vi "Main.vi"() -> ()   [LabVIEW 2026, in "Application.lvlib"]
doc: "This VI is the main application VI in the DQMH project template. This application VI is implemented as a simple state machine, which communicates with two different DQMH modules.\n_____\nBased on DQMH Dev Tools: Project Template 7.1.2.1547."
uses:
  Application.lvlib
  Application Data--cluster.ctl
  State--enum.ctl
  <vilib>/Utility/error.llb/DialogType.ctl
  <vilib>/Utility/error.llb/Search and Replace Pattern (string).vi
  My Cloneable Module/My Cloneable Module.lvlib
  testCoordinator/testCoordinator.lvlib
panel:
  in  "Start Test Procedure":bool
  out "element":string
  in  "Multicolumn Listbox":i32(listbox)
  in  "About DQMH":bool
  out "version":string
  in  "Hide My Singleton Module":bool
  in  "Show My Singleton Module":bool
  in  "Hide My Cloneable Module":bool
  in  "Show My Cloneable Module":bool
  in  "Stop My Cloneable Module":bool
  in  "Stop My Singleton Module":bool
  in  "Start My Singleton Module":bool
  out "Active Cloneable Modules":string[](array[string])
  in  "Start New Instance My Cloneable Module":bool
  in  "Select Cloneable Module Instance":i32(ring)=-1 items=["All"=-1]
  in  "My Singleton Module: Do Something Else":dbl caption="Do Something Else"
  in  "My Singleton Module: Do Something":bool
  out "My Singleton Running?":bool
  out "Status":string
  in  "My Cloneable Module: Do Something Else":dbl caption="Do Something Else to Selected Module"
  in  "My Cloneable Module: Do Something":bool caption="Do Something to Selected Module"
  # "This top-level application allows you to launch and control a singleton module, and multiple instances of a cloneable module."
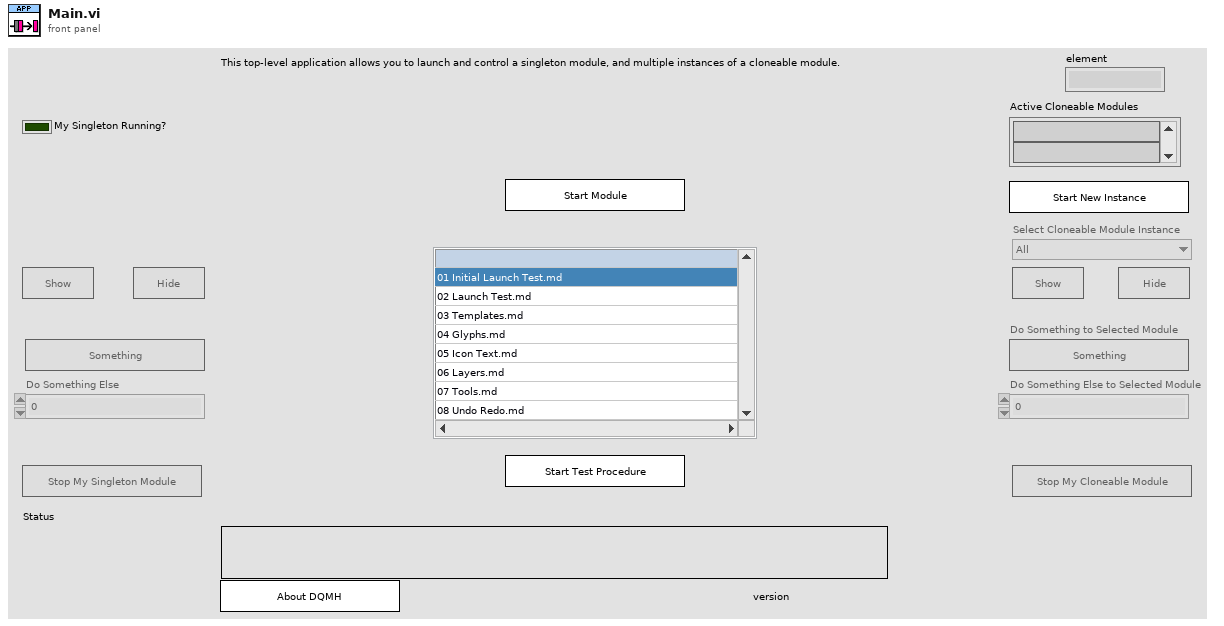
[diagram p1: front panel]
types:
  T1 = typedef "Application.lvlib/State--enum.ctl" = enum16{"Initialize", "Initialize Panel", "UI Interlocks", "Update Status", "Wait for Event", "Exit"}
  T2 = typedef "Application.lvlib/Application Data--cluster.ctl" = cluster{"Status":string, "Singleton Controls":refnum<vi>[], "Cloneable Controls":refnum<vi>[], "Module Ring Value":i32}
  T3 = typedef "My Cloneable Module.lvlib/Broadcast Events--cluster.ctl" = cluster{"Module Did Init":refnum<user-event>, "Status Updated":refnum<user-event>, "Error Reported":refnum<user-event>, "Did Something":refnum<user-event>, "Module Did Stop":refnum<user-event>, "Update Module Execution Status":refnum<user-event>}
  T4 = typedef "testCoordinator.lvlib/Broadcast Events--cluster.ctl" = cluster{"Module Did Init":refnum<user-event>, "Status Updated":refnum<user-event>, "Error Reported":refnum<user-event>, "Did Something":refnum<user-event>, "Module Did Stop":refnum<user-event>, "Update Module Execution Status":refnum<user-event>, "Broadcast Available Tests":refnum<user-event>, "Refresh Test Procedure Indicator":refnum<user-event>, "Refresh Section Indicator":refnum<user-event>, "Refresh Instruction Indicator":refnum<user-event>, "Broadcast Test Scope":refnum<user-event>, "Broadcast Actual Test Procedure Section":refnum<user-event>}
  T5 = enum8{"Enabled", "Disabled", "Disabled and Grayed Out"}
  T6 = typedef "DialogType.ctl" = u16
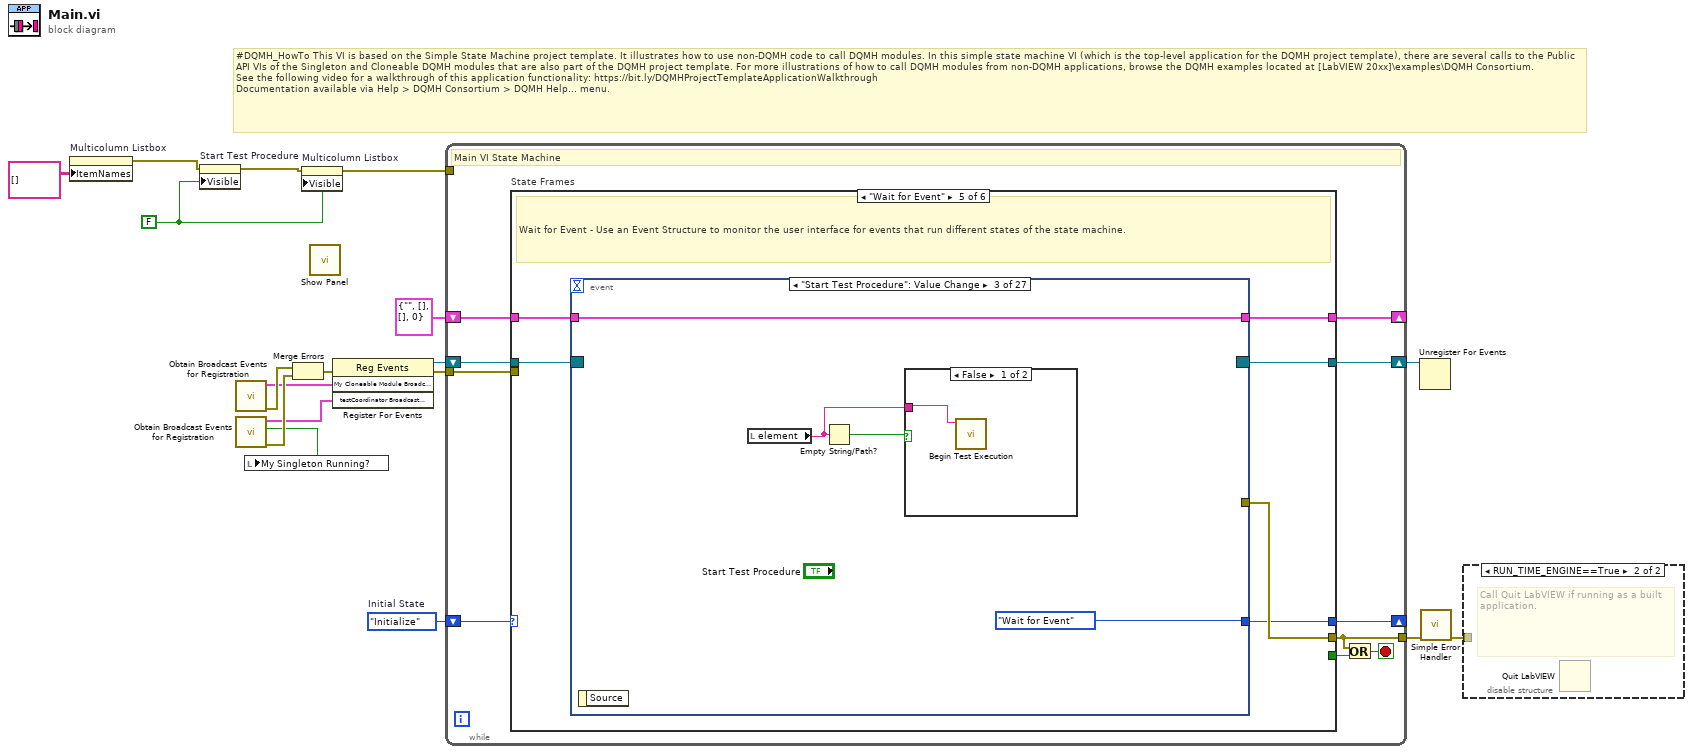
[diagram p0: block diagram]
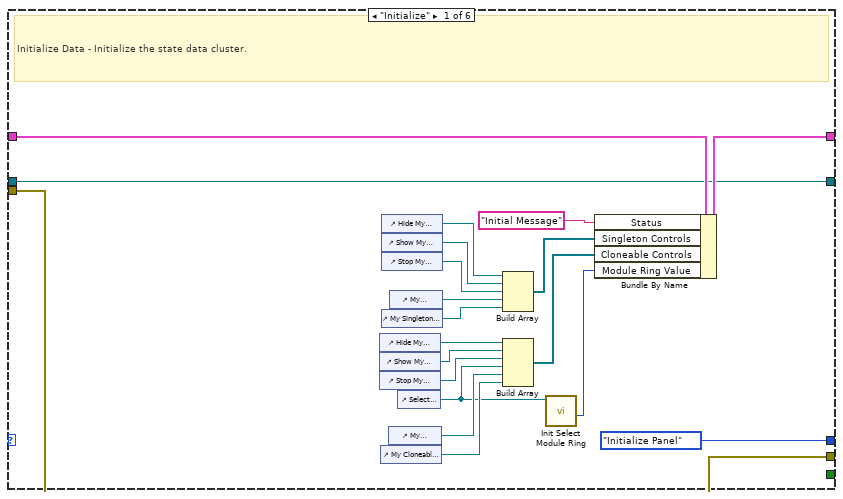
[diagram p2: hidden frame]
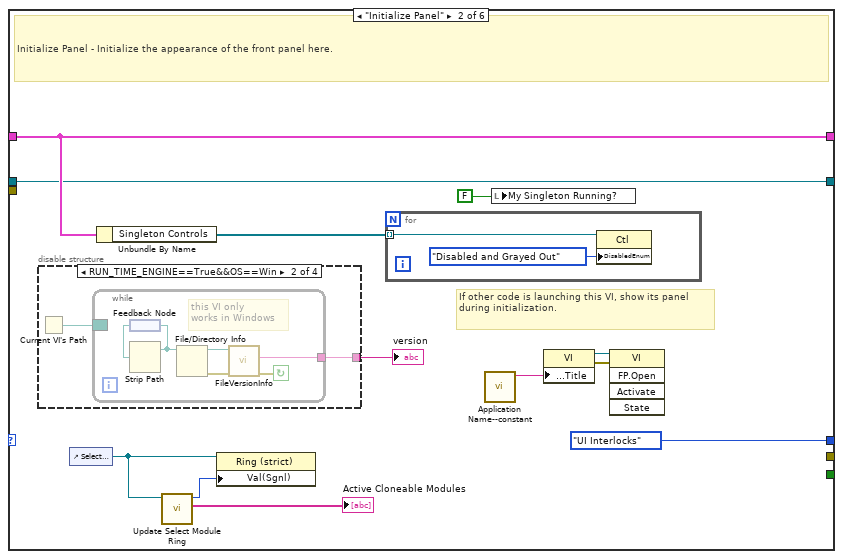
[diagram p3: hidden frame]
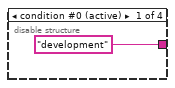
[diagram p4: hidden frame]
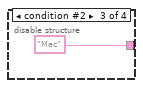
[diagram p5: hidden frame]
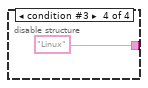
[diagram p6: hidden frame]
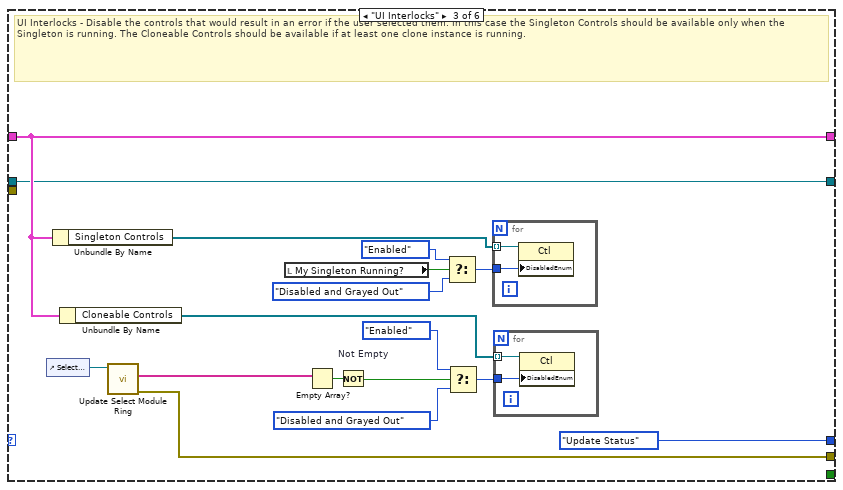
[diagram p7: hidden frame]
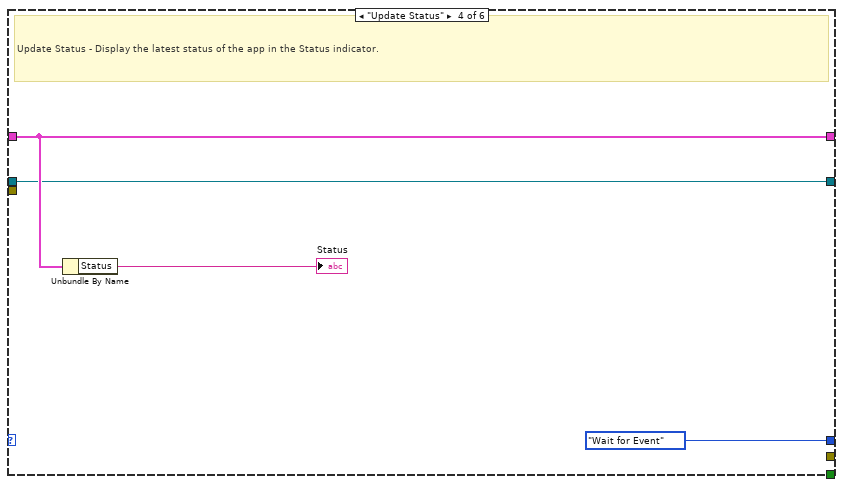
[diagram p8: hidden frame]
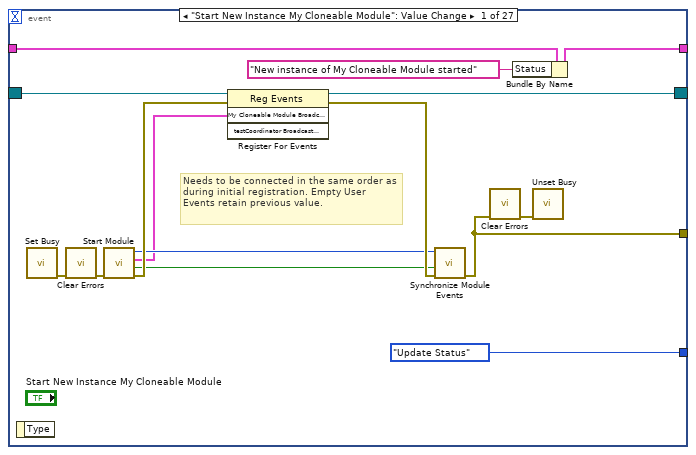
[diagram p9: hidden frame]
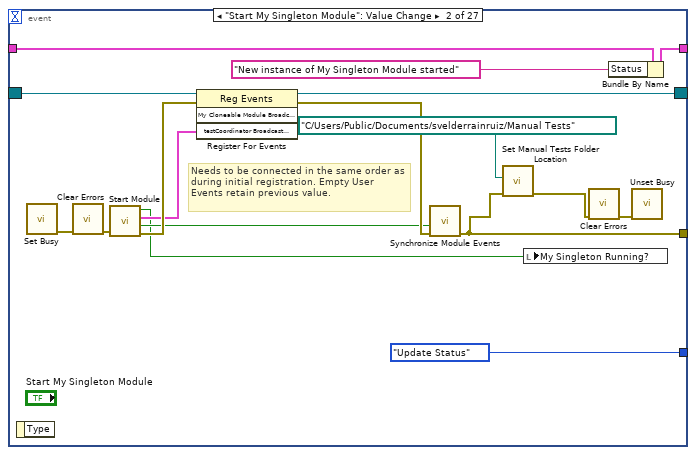
[diagram p10: hidden frame]
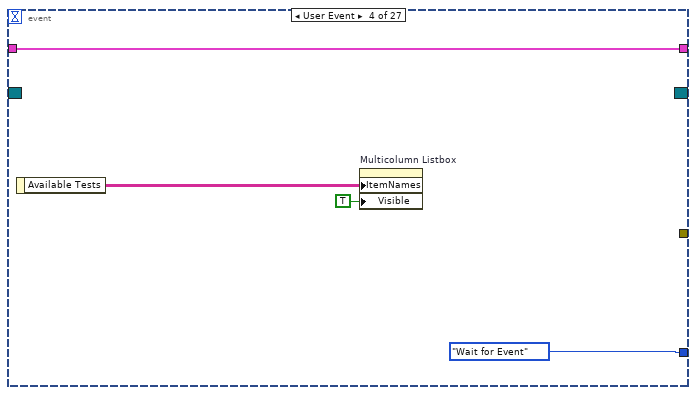
[diagram p12: hidden frame]
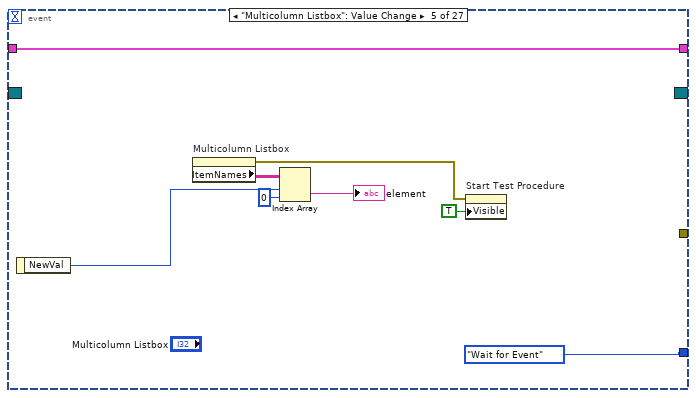
[diagram p13: hidden frame]
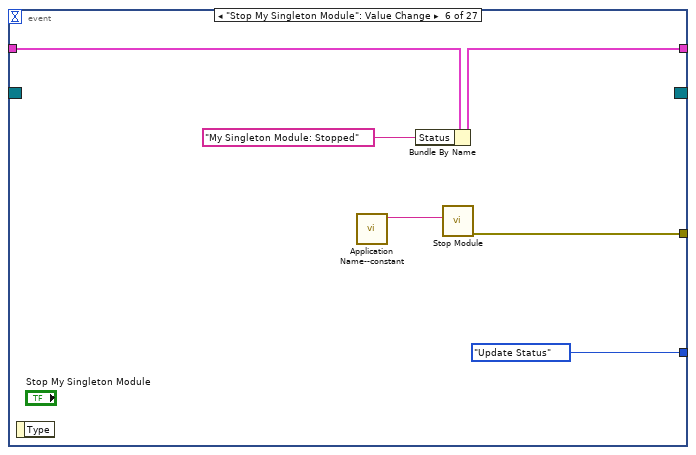
[diagram p14: hidden frame]
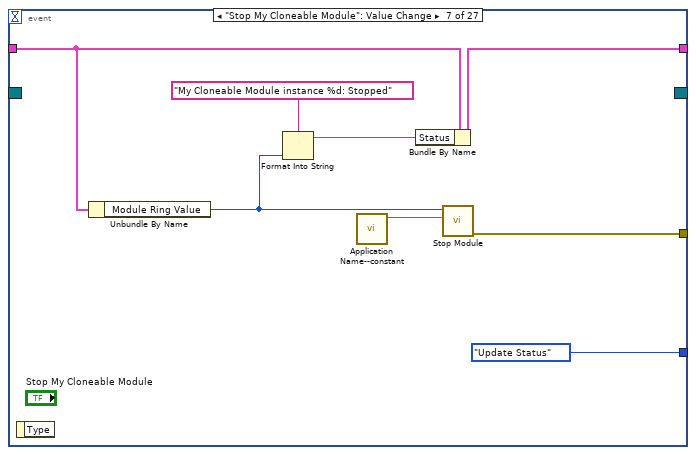
[diagram p15: hidden frame]
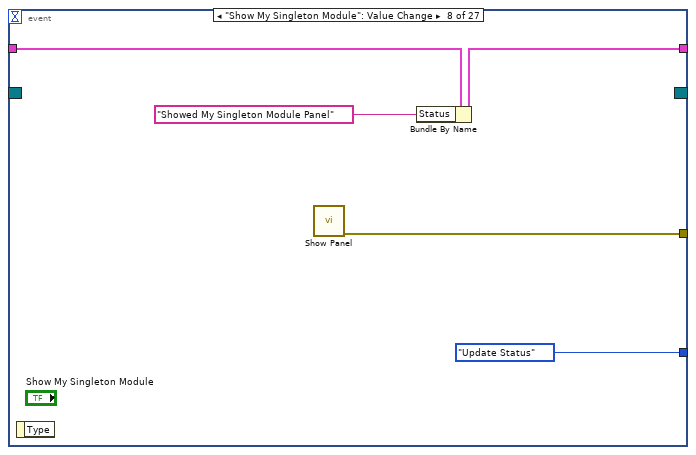
[diagram p16: hidden frame]
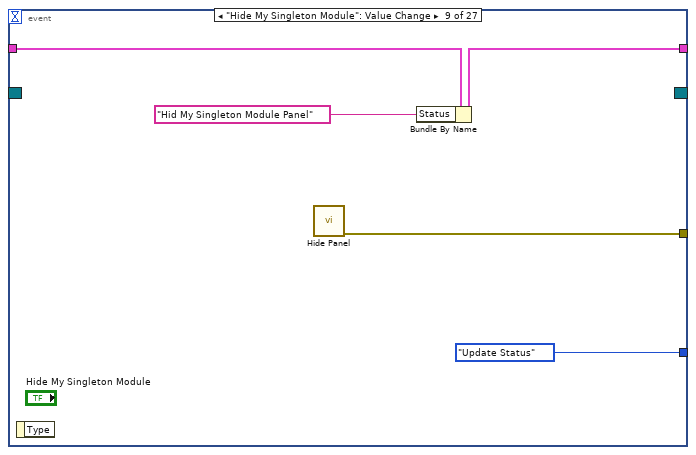
[diagram p17: hidden frame]
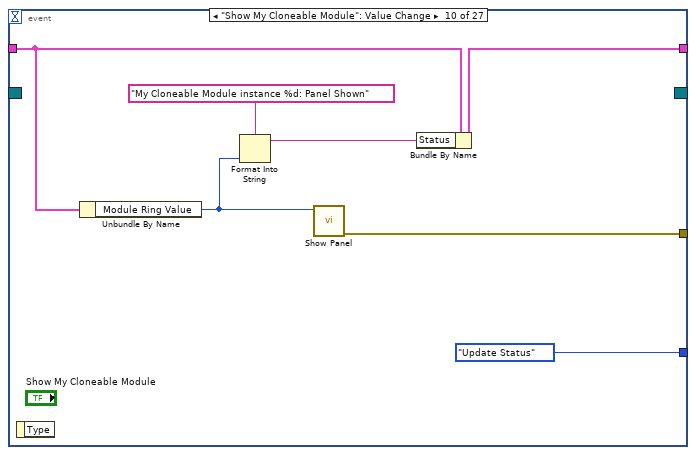
[diagram p18: hidden frame]
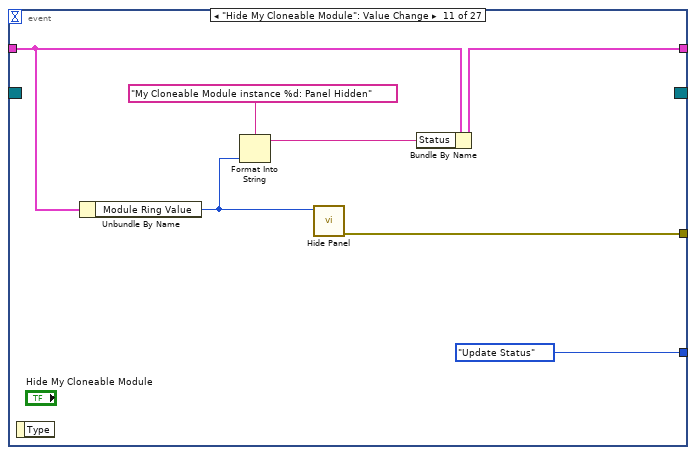
[diagram p19: hidden frame]
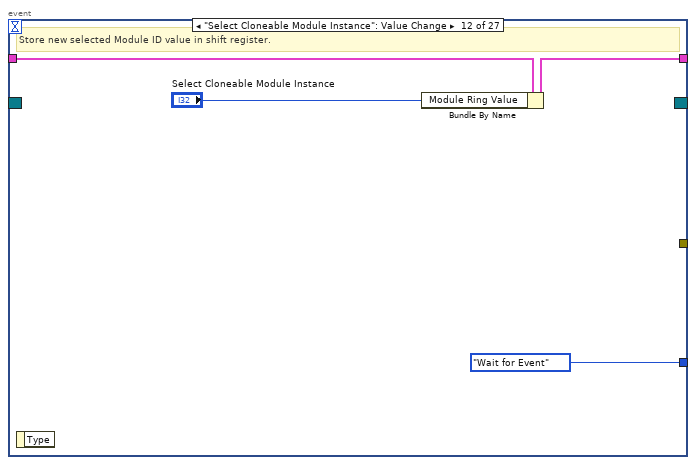
[diagram p20: hidden frame]
diagram:
  w3 = FALSE ("Visible")
  w9 = State--enum."Initialize"  # Initial State
  # "#DQMH_HowTo This VI is based on the Simple State Machine project template. It illustrates how to use non-DQMH code to call DQMH modules. In this simple state machine VI (which is the top-level application for the DQMH project template), there are several calls to the Public API VIs of the Singleton and Cloneable DQMH modules that are also part of the DQMH project template. For more illustrations of how to call DQMH modules from non-DQMH applications, browse the DQMH examples located at [LabVIEW 20xx]\\examples\\DQMH Consortium.\nSee the following video for a walkthrough of this application functionality: https://bit.ly/DQMHProjectTemplateApplicationWalkthrough\nDocumentation available via Help > DQMH Consortium > DQMH Help... menu."
  n1 = property on="Multicolumn Listbox" class="MCListbox (strict)"("ItemNames"=string[][] [] ("Item Names")) -> (error out=w2:errorcluster)  [unwired: 2 in, 1 out]
  n2 = property on="Start Test Procedure" class="Bool"(error in=w2, "Visible"=w3) -> (error out=w4:errorcluster)  [unwired: 1 in, 1 out]
  n3 = call "Obtain Broadcast Events for Registration.vi"() -> ("error out"=w14:errorcluster, "My Cloneable Module Broadcast Events"=w11:T3)  [unwired: 9 in, 1 out]
  n4 = call "Obtain Broadcast Events for Registration.vi"() -> ("error out"=w13:errorcluster, "Already running?"=w6:bool, "testCoordinator Broadcast Events"=w10:T4)  [unwired: 9 in]
  n5 = local write "My Singleton Running?"(w6) -> ()
  n6 = Merge Errors(w14, w13) -> (w15:errorcluster)
  n7 = property on="Multicolumn Listbox" class="MCListbox (strict)"(error in=w4, "Visible"=w3) -> (error out=w5:errorcluster)  [unwired: 1 in, 1 out]
  n8 = call "Show Panel.vi"() -> ()  [unwired: 11 in, 1 out]
  n9 = register-events(error in=w15, w11, w10) -> (reference out=w8:refnum<event-registration>, error out=w16:errorcluster)  [unwired: 1 in]
  n10 = while {
    shift-right: [w25] -> _
    shift-left: T2 {"Status"="", "Singleton Controls"=[], "Cloneable Controls"=[], "Module Ring Value"=0} ("Data Cluster") -> [w26]
    tunnel: [w28] -> w18
    shift-right: [w21] -> _
    shift-left: w9 -> [w23]
    shift-right: [w19] -> w7
    shift-left: w8 -> [w20]
    tunnel: w16 -> [w27]
    tunnel: w5 -> [_]
    stop <- w22 stop-if-true
    # "Main VI State Machine"
    n11 = case "State Frames" shown="\"Wait for Event\"" w23 {
      tunnel: [w48 _ w90 _ w104 w301] -> w28
      tunnel: w26 -> [w47 w57 w78 w98 w101 w298]
      tunnel: [w46 w57 w78 w98 w100 w298] -> w25
      tunnel: [_ _ _ _ _ w297] -> w24
      tunnel: [State--enum."Initialize Panel" ("State") State--enum."UI Interlocks" ("State") State--enum."Update Status" ("State") State--enum."Wait for Event" ("State") w99 State--enum."Exit" ("State")] -> w21
      tunnel: w20 -> [w29 w54 w74 w95 w103 w295]
      tunnel: [w29 w54 w74 w95 w102 w295] -> w19
      tunnel: w27 -> [w48 _ _ _ _ _]
      frame "Initialize" {
        # "Initialize Data - Initialize the state data cluster."
        n12 = control-ref of="Hide My Cloneable Module"() -> (w38:refnum<vi>)
        n13 = control-ref of="Show My Cloneable Module"() -> (w37:refnum<vi>)
        n14 = control-ref of="Stop My Cloneable Module"() -> (w36:refnum<vi>)
        n15 = control-ref of="My Cloneable Module: Do Something"() -> (w33:refnum<vi>)
        n16 = control-ref of="Hide My Singleton Module"() -> (w44:refnum<vi>)
        n17 = control-ref of="Show My Singleton Module"() -> (w43:refnum<vi>)
        n18 = control-ref of="Stop My Singleton Module"() -> (w42:refnum<vi>)
        n19 = control-ref of="My Singleton Module: Do Something"() -> (w40:refnum<vi>)
        n20 = control-ref of="My Cloneable Module: Do Something Else"() -> (w34:refnum<vi>)
        n21 = control-ref of="My Singleton Module: Do Something Else"() -> (w41:refnum<vi>)
        n22 = control-ref of="Select Cloneable Module Instance"() -> (w31:refnum<vi>)
        n23 = Build Array(w44, w43, w42, w41, w40) -> (w39:refnum<vi>[])
        n24 = Build Array(w38, w37, w36, w31, w34, w33) -> (w35:refnum<vi>[])
        n25 = call "Init Select Module Ring.vi"("Select Module Ring Ref"=w31) -> ("Module Ring Value"=w30:i32)  [unwired: 8 in, 2 out]
        n26 = Bundle By Name(cluster=w47, "Status"="Initial Message" ("Initial Message"), "Singleton Controls"=w39, "Cloneable Controls"=w35, "Module Ring Value"=w30) -> (w46:T2)
      }
      frame "Initialize Panel" {
        # "If other code is launching this VI, show its panel during initialization."
        # "Initialize Panel - Initialize the appearance of the front panel here."
        n27 = disable-structure "Conditional Disable Structure" shown="RUN_TIME_ENGINE==True&&OS==Win" {
          disable-tunnel: ["development" w62 "Mac" "Linux"] -> w51
          frame condition #0 (active) {
          }
          frame condition #1 {
            n28 = Current VI's Path() -> (path=w63:path)
            n29 = while {
              border: w63 -> [_]
              tunnel: [w64] -> w62
              stop <- w68 continue-if-true
              # "this VI only \nworks in Windows"
              n30 = feedback #1() -> (w67:path)
              n31 = Strip Path(path=w67) -> (stripped path=w66:path)  [unwired: 1 out]
              n32 = feedback-in #1(w66) -> ()
              n33 = File/Directory Info(path=w66) -> (path out=w65:path, error out=w69:errorcluster)  [unwired: 1 in, 5 out]
              n34 = call <vilib>:"FileVersionInfo.vi"("error in (no error)"=w69, "Application Path in"=w65) -> ("error out"=w68:errorcluster, "File Version Info"=w64:string)  [unwired: 6 in, 2 out]
            }
          }
          frame condition #2 {
          }
          frame condition #3 {
          }
        }
        "version" <- w51
        n35 = control-ref of="Select Cloneable Module Instance"() -> (w53:refnum<vi>)
        n36 = Unbundle By Name(w57) -> ("Singleton Controls"=w56:refnum<vi>[])
        n37 = call "Update Select Module Ring.vi"("Select Module Ring Ref"=w53) -> ("Active Modules (Array)"=→"Active Cloneable Modules":string[], "New Module Ring Value"=w52:i32)  [unwired: 8 in, 1 out]
        n38 = property on="Property Node" class="Ring (strict)"(reference=w53, "Val(Sgnl)"=w52) -> ()  [unwired: 1 in, 2 out]
        n39 = for {
          tunnel: w56 -> [w73] mode=indexing
          n40 = property on="Property Node" class="Ctl"(reference=w73, "DisabledEnum"=T5."Disabled and Grayed Out" ("Disabled")) -> ()  [unwired: 1 in, 2 out]
        }
        n41 = call "Application Name--constant.vi"() -> ("Application Name"=w50:string)  [unwired: 11 in]
        n42 = local write "My Singleton Running?"(FALSE ("My Singleton Module Init?")) -> ()
        n43 = property on="Property Node" class="VI"("Front Panel.Title"=w50) -> (reference out=w49:refnum<vi>, error out=w60:errorcluster)  [unwired: 2 in]
        n44 = invoke class="VI" method="FP.Open"(reference=w49, error in=w60) -> ()  [unwired: 3 in, 5 out]
      }
      frame "UI Interlocks" {
        # "UI Interlocks - Disable the controls that would result in an error if the user selected them. In this case the Singleton Controls should be available only when the Singleton is running. The Cloneable Controls should be available if at least one clone instance is running."
        n45 = control-ref of="Select Cloneable Module Instance"() -> (w89:refnum<vi>)
        n46 = Unbundle By Name(w78) -> ("Singleton Controls"=w83:refnum<vi>[])
        n47 = Unbundle By Name(w78) -> ("Cloneable Controls"=w77:refnum<vi>[])
        n48 = call "Update Select Module Ring.vi"("Select Module Ring Ref"=w89) -> ("error out"=w90:errorcluster, "Active Modules (Array)"=w88:string[])  [unwired: 8 in, 1 out]
        n49 = local read "My Singleton Running?"() -> (w82:bool)
        n50 = Empty Array?(array=w88) -> (empty?=w87:bool)
        n51 = Not "Not Empty"(x=w87) -> (.not. x?=w76:bool)
        n52 = Select(t=T5."Enabled" ("Disabled"), s=w82, f=T5."Disabled and Grayed Out" ("Disabled")) -> (s? t:f=w84:T5)
        n53 = Select(t=T5."Enabled" ("Disabled"), s=w76, f=T5."Disabled and Grayed Out" ("Disabled")) -> (s? t:f=w81:T5)
        n54 = for {
          tunnel: w83 -> [w94] mode=indexing
          tunnel: w84 -> [w93]
          n55 = property on="Property Node" class="Ctl"(reference=w94, "DisabledEnum"=w93) -> ()  [unwired: 1 in, 2 out]
        }
        n56 = for {
          tunnel: w77 -> [w92] mode=indexing
          tunnel: w81 -> [w91]
          n57 = property on="Property Node" class="Ctl"(reference=w92, "DisabledEnum"=w91) -> ()  [unwired: 1 in, 2 out]
        }
      }
      frame "Update Status" {
        # "Update Status - Display the latest status of the app in the Status indicator."
        n58 = Unbundle By Name(w98) -> ("Status"=→"Status":string)
      }
      frame "Wait for Event" {
        # "Wait for Event - Use an Event Structure to monitor the user interface for events that run different states of the state machine."
        n59 = event shown="[2] \"Start Test Procedure\": Value Change" {
          selector: w103 -> [w111 w130 _ _ _ _ _ _ _ _ _ _ _ _ _ _ _ _ _ _ _ _ _ _ _ _ _]
          dyn-events: [w110 w129 _ _ _ _ _ _ _ _ _ _ _ _ _ _ _ _ _ _ _ _ _ _ _ _ _] -> w102
          timeout: _ -> [_ _ _ _ _ _ _ _ _ _ _ _ _ _ _ _ _ _ _ _ _ _ _ _ _ _ _]
          tunnel: [w119 w121 _ _ _ w159 w167 w172 w177 w184 w191 _ w200 w206 w212 w219 w227 w232 w236 _ _ _ _ w278 _ _ w289] -> w104
          tunnel: [w106 w126 w140 w145 w153 w155 w164 w170 w175 w183 w190 w193 w198 w205 w210 w218 w221 w229 w235 w238 w243 w258 w267 w271 w282 w287 w291] -> w100
          tunnel: w101 -> [w107 w127 w140 w145 w153 w156 w163 w171 w176 w181 w188 w194 w199 w202 w211 w216 w221 w229 w235 w239 w244 w259 w268 w274 w283 w287 w291]
          tunnel: [State--enum."Update Status" ("State") State--enum."Update Status" ("State") State--enum."Wait for Event" ("State") State--enum."Wait for Event" ("State") State--enum."Wait for Event" ("State") State--enum."Update Status" ("State") State--enum."Update Status" ("State") State--enum."Update Status" ("State") State--enum."Update Status" ("State") State--enum."Update Status" ("State") State--enum."Update Status" ("State") State--enum."Wait for Event" ("State") State--enum."Wait for Event" ("State") State--enum."Wait for Event" ("State") State--enum."Update Status" ("State") State--enum."Update Status" ("State") State--enum."UI Interlocks" ("State") State--enum."UI Interlocks" ("State") State--enum."UI Interlocks" ("State") State--enum."Update Status" ("State") State--enum."Update Status" ("State") State--enum."Update Status" ("State") State--enum."Update Status" ("State") State--enum."UI Interlocks" ("State") State--enum."UI Interlocks" ("State") State--enum."Exit" ("State") State--enum."Wait for Event" ("State")] -> w99
          event "Start New Instance My Cloneable Module": Value Change {
            # "Needs to be connected in the same order as during initial registration. Empty User Events retain previous value."
            n60 = event-data() -> ()  [unwired: 1 in, 1 out]
            n61 = call <vilib>:"Set Busy.vi"() -> ("error out"=w115:errorcluster)  [unwired: 10 in, 1 out]
            n62 = call <vilib>:"Clear Errors.vi"("error in (no error)"=w115) -> ("error out"=w116:errorcluster)  [unwired: 5 in, 1 out]
            n63 = call "Start Module.vi"("error in"=w116) -> ("error out"=w118:errorcluster, "Wait for Event Sync?"=w113:bool, "My Cloneable Module Broadcast Events"=w109:T3, "Module ID"=w112:i32)  [unwired: 6 in, 1 out]
            n64 = register-events(reference=w111, error in=w118, w109) -> (reference out=w110:refnum<event-registration>, error out=w117:errorcluster)  [unwired: 1 in]
            n65 = call "Synchronize Module Events.vi"("error in"=w117, "Wait for Event Sync?"=w113, "Module ID in"=w112) -> ("error out"=w119:errorcluster)  [unwired: 7 in, 1 out]
            n66 = call <vilib>:"Clear Errors.vi"("error in (no error)"=w119) -> ("error out"=w114:errorcluster)  [unwired: 5 in, 1 out]
            n67 = Bundle By Name(cluster=w107, "Status"="New instance of My Cloneable Module started") -> (w106:T2)
            n68 = call <vilib>:"Unset Busy.vi"("error in (no error)"=w114) -> ()  [unwired: 10 in, 1 out]
          }
          event "Start My Singleton Module": Value Change {
            # "Needs to be connected in the same order as during initial registration. Empty User Events retain previous value."
            n69 = event-data() -> ()  [unwired: 1 in, 1 out]
            n70 = call <vilib>:"Set Busy.vi"() -> ("error out"=w133:errorcluster)  [unwired: 10 in, 1 out]
            n71 = call <vilib>:"Clear Errors.vi"("error in (no error)"=w133) -> ("error out"=w134:errorcluster)  [unwired: 5 in, 1 out]
            n72 = call "Start Module.vi"("error in"=w134) -> ("error out"=w136:errorcluster, "Wait for Event Sync?"=w131:bool, "testCoordinator Broadcast Events"=w124:T4, "Module Was Already Running?"=w123:bool)  [unwired: 6 in, 1 out]
            n73 = register-events(reference=w130, error in=w136, w124) -> (reference out=w129:refnum<event-registration>, error out=w135:errorcluster)  [unwired: 1 in]
            n74 = call "Synchronize Module Events.vi"("error in"=w135, "Wait for Event Sync?"=w131) -> ("error out"=w121:errorcluster)  [unwired: 9 in]
            n75 = call "Set Manual Tests Folder Location.vi"("error in"=w121, "Manual Tests Folder"=path "C:/Users/Public/Documents/svelderrainruiz/Manual Tests") -> ("error out"=w120:errorcluster)  [unwired: 7 in, 2 out]
            n76 = local write "My Singleton Running?"(w123) -> ()
            n77 = call <vilib>:"Clear Errors.vi"("error in (no error)"=w120) -> ("error out"=w132:errorcluster)  [unwired: 5 in, 1 out]
            n78 = Bundle By Name(cluster=w127, "Status"="New instance of My Singleton Module started") -> (w126:T2)
            n79 = call <vilib>:"Unset Busy.vi"("error in (no error)"=w132) -> ()  [unwired: 10 in, 1 out]
          }
          event "Start Test Procedure": Value Change {
            n80 = event-data() -> ()  [unwired: 1 in, 1 out]
            n81 = local read "element"() -> (w138:string)
            n82 = Empty String/Path?(string/path=w138) -> (empty?=w139:bool)
            n83 = case shown="False" w139 {
              tunnel: w138 -> [w141 _]
              frame False {
                n84 = call "Begin Test Execution.vi"("Test Procedure"=w141) -> ()  [unwired: 10 in, 1 out]
              }
              frame True {
              }
            }
          }
          event User Event {
            n85 = event-data() -> ("Available Tests"=w144:string[][])  [unwired: 1 in]
            n86 = property on="Multicolumn Listbox" class="MCListbox (strict)"("ItemNames"=w144, "Visible"=TRUE) -> ()  [unwired: 2 in, 2 out]
          }
          event "Multicolumn Listbox": Value Change {
            n87 = event-data() -> ("NewVal"=w151:i32)  [unwired: 1 in]
            n88 = property on="Multicolumn Listbox" class="MCListbox (strict)"() -> (error out=w146:errorcluster, "ItemNames"=w152:string[][])  [unwired: 2 in, 1 out]
            n89 = Index Array(array=w152, index (row)=w151, index (col)=0 ("disabled index (col)")) -> (element=→"element":string)
            n90 = property on="Start Test Procedure" class="Bool"(error in=w146, "Visible"=TRUE) -> ()  [unwired: 1 in, 2 out]
          }
          event "Stop My Singleton Module": Value Change {
            n91 = event-data() -> ()  [unwired: 1 in, 1 out]
            n92 = call "Application Name--constant.vi"() -> ("Application Name"=w157:string)  [unwired: 11 in]
            n93 = Bundle By Name(cluster=w156, "Status"="My Singleton Module: Stopped" ("Message")) -> (w155:T2)
            n94 = call "Stop Module.vi"("Origin"=w157) -> ("error out"=w159:errorcluster)  [unwired: 10 in]
          }
          event "Stop My Cloneable Module": Value Change {
            n95 = event-data() -> ()  [unwired: 1 in, 1 out]
            n96 = Unbundle By Name(w163) -> ("Module Ring Value"=w160:i32)
            n97 = Format Into String(format string="My Cloneable Module instance %d: Stopped" ("Message"), w160) -> (resulting string=w161:string)  [unwired: 2 in, 1 out]
            n98 = call "Application Name--constant.vi"() -> ("Application Name"=w165:string)  [unwired: 11 in]
            n99 = Bundle By Name(cluster=w163, "Status"=w161) -> (w164:T2)
            n100 = call "Stop Module.vi"("Origin"=w165, "Module ID"=w160) -> ("error out"=w167:errorcluster)  [unwired: 9 in]
          }
          event "Show My Singleton Module": Value Change {
            n101 = event-data() -> ()  [unwired: 1 in, 1 out]
            n102 = call "Show Panel.vi"() -> ("error out"=w172:errorcluster)  [unwired: 11 in]
            n103 = Bundle By Name(cluster=w171, "Status"="Showed My Singleton Module Panel" ("Message")) -> (w170:T2)
          }
          event "Hide My Singleton Module": Value Change {
            n104 = event-data() -> ()  [unwired: 1 in, 1 out]
            n105 = call "Hide Panel.vi"() -> ("error out"=w177:errorcluster)  [unwired: 11 in]
            n106 = Bundle By Name(cluster=w176, "Status"="Hid My Singleton Module Panel" ("Message")) -> (w175:T2)
          }
          event "Show My Cloneable Module": Value Change {
            n107 = event-data() -> ()  [unwired: 1 in, 1 out]
            n108 = Unbundle By Name(w181) -> ("Module Ring Value"=w179:i32)
            n109 = Format Into String(format string="My Cloneable Module instance %d: Panel Shown" ("Message"), w179) -> (resulting string=w178:string)  [unwired: 2 in, 1 out]
            n110 = call "Show Panel.vi"("Module ID"=w179) -> ("error out"=w184:errorcluster)  [unwired: 10 in]
            n111 = Bundle By Name(cluster=w181, "Status"=w178) -> (w183:T2)
          }
          event "Hide My Cloneable Module": Value Change {
            n112 = event-data() -> ()  [unwired: 1 in, 1 out]
            n113 = Unbundle By Name(w188) -> ("Module Ring Value"=w186:i32)
            n114 = Format Into String(format string="My Cloneable Module instance %d: Panel Hidden" ("Message"), w186) -> (resulting string=w185:string)  [unwired: 2 in, 1 out]
            n115 = call "Hide Panel.vi"("Module ID"=w186) -> ("error out"=w191:errorcluster)  [unwired: 10 in]
            n116 = Bundle By Name(cluster=w188, "Status"=w185) -> (w190:T2)
          }
          event "Select Cloneable Module Instance": Value Change {
            # "Store new selected Module ID value in shift register."
            n117 = event-data() -> ()  [unwired: 1 in, 1 out]
            n118 = Bundle By Name(cluster=w194, "Module Ring Value"="Select Cloneable Module Instance") -> (w193:T2)
          }
          event "My Singleton Module: Do Something": Value Change {
            w197 = "\"Something\" button pressed in top-level application VI" ("\"Do Something Else\" button pressed")
            # "Send \"Do Something\" request to My Singleton Module"
            n119 = event-data() -> ()  [unwired: 1 in, 1 out]
            n120 = call "Do Something.vi"("Do Something Message"=w197) -> ("error out"=w200:errorcluster)  [unwired: 10 in]
            n121 = Bundle By Name(cluster=w199, "Status"=w197) -> (w198:T2)
          }
          event "My Cloneable Module: Do Something": Value Change {
            w204 = "\"Something\" button pressed in top-level application VI" ("\"Do Something Else\" button pressed")
            # "Send \"Do Something\" request to My Cloneable Module"
            n122 = event-data() -> ()  [unwired: 1 in, 1 out]
            n123 = Unbundle By Name(w202) -> ("Module Ring Value"=w201:i32)
            n124 = call "Do Something.vi"("Do Something Message"=w204, "Module ID"=w201) -> ("error out"=w206:errorcluster)  [unwired: 9 in]
            n125 = Bundle By Name(cluster=w202, "Status"=w204) -> (w205:T2)
          }
          event "My Singleton Module: Do Something Else": Value Change {
            w207 = "\"Do Something Else\" numeric value changed in top-level application VI. New value: " ("\"Do Something Else\" button pressed")
            # "Send \"Do Something Else\" request to My Singleton Module"
            n126 = event-data() -> ()  [unwired: 1 in, 1 out]
            n127 = call "Do Something Else.vi"("X"="My Singleton Module: Do Something Else", "Do Something Else Message"=w207) -> ("error out"=w212:errorcluster)  [unwired: 9 in]
            n128 = Bundle By Name(cluster=w211, "Status"=w207) -> (w210:T2)
          }
          event "My Cloneable Module: Do Something Else": Value Change {
            w213 = "\"Do Something Else\" numeric value changed in top-level application VI. New value: " ("\"Do Something Else\" button pressed")
            # "Send \"Do Something Else\" request to My Cloneable Module"
            n129 = event-data() -> ()  [unwired: 1 in, 1 out]
            n130 = Unbundle By Name(w216) -> ("Module Ring Value"=w215:i32)
            n131 = call "Do Something Else.vi"("X"="My Cloneable Module: Do Something Else", "Do Something else Message"=w213, "Module ID"=w215) -> ("error out"=w219:errorcluster)  [unwired: 8 in]
            n132 = Bundle By Name(cluster=w216, "Status"=w213) -> (w218:T2)
          }
          event User Event {
            # "A new instance of My Cloneable Module has broadcast that is has been initialized"
            n133 = event-data() -> ("Info"=w225:string, "Module ID"=w220:i32)  [unwired: 1 in]
            n134 = local write "Status"(w225) -> ()
            n135 = control-ref of="Select Cloneable Module Instance"() -> (w224:refnum<vi>)
            n136 = call "Update Select Module Ring.vi"("Select Module Ring Ref"=w224) -> ("error out"=w226:errorcluster, "Active Modules (Array)"=w223:string[])  [unwired: 8 in, 1 out]
            n137 = local write "Active Cloneable Modules"(w223) -> ()
            n138 = call "Show Panel.vi"("error in"=w226, "Module ID"=w220) -> ("error out"=w227:errorcluster)  [unwired: 9 in]
          }
          event User Event {
            # "My Singleton Module has broadcast that it has been initialized"
            n139 = event-data() -> ("Init?"=→"My Singleton Running?":bool, "Info"=w231:string)  [unwired: 1 in]
            n140 = local write "Status"(w231) -> ()
            n141 = call "Show Panel.vi"() -> ("error out"=w232:errorcluster)  [unwired: 11 in]
          }
          event User Event {
            # "My Singleton Module has broadcast its execution status"
            n142 = event-data() -> ("Running?"=w233:bool)  [unwired: 1 in]
            n143 = local write "My Singleton Running?"(w233) -> ()
            n144 = case shown="True" w233 {
              tunnel: [_ w237] -> w236
              frame False {
              }
              frame True {
                n145 = call "Show Panel.vi"() -> ("error out"=w237:errorcluster)  [unwired: 11 in]
              }
            }
          }
          event User Event {
            # "An instance of My Cloneable Module has broadcast its status"
            n146 = event-data() -> ("Status"=w241:string)  [unwired: 1 in]
            n147 = Bundle By Name(cluster=w239, "Status"=w241) -> (w238:T2)
          }
          event User Event {
            # "My Singleton Module has broadcast its status"
            n148 = event-data() -> ("Status"=w245:string)  [unwired: 1 in]
            n149 = Bundle By Name(cluster=w244, "Status"=w245) -> (w243:T2)
          }
          event User Event {
            w250 = T6 0 items=["no dialog", "OK message", "continue or stop message", "OK message + warnings", "continue/stop + warnings"] ("type of dialog (OK msg:1)")
            # "My Cloneable Module had an error"
            n150 = event-data() -> ("Module Name"=w247:string, "Additional Information"=w248:string, "Error"=w249:errorcluster)  [unwired: 1 in]
            n151 = call <vilib>:"Space Constant.vi"() -> ("String"=w254:string)
            n152 = call <vilib>:"Simple Error Handler.vi"("type of dialog (OK msg:1)"=w250, "error in (no error)"=w249) -> ("message"=w251:string)  [unwired: 3 in, 4 out]
            n153 = call-poly <vilib>:"Search and Replace Pattern.vi"("string"=w251, "regular expression (\"\")"="[\\r\\n]" ("regular expression (\"\")"), "replace string (\"\")"=w254, "replace all? (F)"=TRUE ("replace all CR/LF with spaces")) -> ("result string"=w252:string)  [unwired: 1 in, 1 out]
            n154 = Format Into String(format string="%s: %s Additional Information: %s", w247, w252, w248) -> (resulting string=w246:string)  [unwired: 2 in, 1 out]
            n155 = Bundle By Name(cluster=w259, "Status"=w246) -> (w258:T2)
          }
          event User Event {
            # "My Singleton Module had an error"
            n156 = event-data() -> ("Module Name"=w261:string, "Additional Information"=w265:string, "Error"=w269:errorcluster)  [unwired: 1 in]
            n157 = Unbundle By Name(w269) -> ("code"=w260:i32, "source"=w264:string)
            n158 = Format Into String(format string="Error code %d Module: %s  Additional Information: %s\nSource: %s", w260, w261, w265, w264) -> (resulting string=w262:string)  [unwired: 2 in, 1 out]
            n159 = Bundle By Name(cluster=w268, "Status"=w262) -> (w267:T2)
          }
          event User Event {
            n160 = event-data() -> ("Origin"=w273:string)  [unwired: 1 in]
            n161 = Bundle By Name(cluster=w274, "Status"=w273) -> (w272:T2)
            n162 = control-ref of="Select Cloneable Module Instance"() -> (w277:refnum<vi>)
            n163 = call "Update Select Module Ring.vi"("Select Module Ring Ref"=w277) -> ("error out"=w278:errorcluster, "Active Modules (Array)"=w276:string[], "New Module Ring Value"=w270:i32)  [unwired: 8 in]
            n164 = Bundle By Name(cluster=w272, "Module Ring Value"=w270) -> (w271:T2)
            n165 = local write "Active Cloneable Modules"(w276) -> ()
          }
          event User Event {
            n166 = event-data() -> ("Origin"=w280:string)  [unwired: 1 in]
            n167 = local write "My Singleton Running?"(FALSE ("My Singleton Module Init?")) -> ()
            n168 = Concatenate Strings(w280, " Did Stop.") -> (w279:string)
            n169 = Bundle By Name(cluster=w283, "Status"=w279) -> (w282:T2)
          }
          event Panel Close? {
            # "Go to the 'Exit' state if the user tries to close the panel."
            n170 = event-data() -> ()  [unwired: 1 in, 1 out]
            n171 = event-data ("Event Filter Node")("Discard?"=TRUE) -> ()  [unwired: 1 in, 1 out]
          }
          event "About DQMH": Value Change {
            # "Display DQMH About Box"
            n172 = event-data() -> ()  [unwired: 1 in, 1 out]
            n173 = call <vilib>:"DQMH_About Box.vi"() -> ("error out"=w289:errorcluster)  [unwired: 11 in]
          }
        }
      }
      frame "Exit" {
        w292 = TRUE  # Wait for Module to stop?
        w297 = TRUE  # Stop the VI
        # "Stop all modules launched"
        # "Exit - Exit the application."
        n174 = call "Application Name--constant.vi"() -> ("Application Name"=w293:string)  [unwired: 11 in]
        n175 = call "Stop Module.vi"("Wait for Module to stop? (F)"=w292, "Origin"=w293, "Module ID"=-1) -> ("error out"=w299:errorcluster)  [unwired: 8 in]
        n176 = call "Stop Module.vi"("Wait for Module to Stop? (F)"=w292, "Origin"=w293) -> ("error out"=w300:errorcluster)  [unwired: 9 in]
        n177 = Merge Errors(w299, w300) -> (w301:errorcluster)
      }
    }
    n178 = Or(x=w28, y=w24) -> (x .or. y?=w22:bool)
  }
  n179 = Unregister For Events(event registration refnum=w7) -> ()  [unwired: 1 in, 1 out]
  n180 = call <vilib>:"Simple Error Handler.vi"("error in (no error)"=w18) -> ("error out"=w17:errorcluster)  [unwired: 4 in, 4 out]
  n181 = disable-structure "Conditional Disable Structure" shown="RUN_TIME_ENGINE==True" {
    disable-tunnel: w17 -> [_ _]
    frame condition #0 (active) {
    }
    frame condition #1 {
      # "Call Quit LabVIEW if running as a built application."
      n182 = Quit LabVIEW() -> ()  [unwired: 1 in]
    }
  }
